vi "LTE_Example.vi"() -> ()   [LabVIEW 2016]
doc: "This example illustrates how to use the RFmxLTE APIs to configure the analyzer to do ModAcc measurement. You can use the Generator Basic example to generate the LTE signal before running this example."
uses:
  Source/SA/RFmxLTE/Typedefs/LTE ModAcc Configuration.ctl
  Source/SA/RFmxLTE/Typedefs/LTE ModAcc Results.ctl
  Source/SA/RFmxLTE/Typedefs/LTE ModAcc Component Carrier Results.ctl
  Source/SA/RFmxInstr/Typedefs/Instrument Configuration.ctl
  Source/Common/Local Oscillator Sharing Mode.ctl
  Source/Common/SA Common Configuration.ctl
  Source/SA/RFmxLTE/Typedefs/LTE Standard Configuration.ctl
  Source/SA/RFmxLTE/Typedefs/LTE Component Carrier Configuration.ctl
  Source/Common/SA Auto Level Configuration.ctl
  Source/SA/RFmxLTE/RFmxLTE.lvlib
  Source/SA/RFmxInstr/RFmxInstr.lvlib
  Source/Common/Common.lvlib
panel:
  out "error out":errorcluster
  out "ModAcc Results":T1
  in  "Tab Control":enum32{"Common", "Standard", "ModAcc"}(tab)
  in  "Resource Name":refnum<k15>="5840"
  in  "Common Configuration":T3={"Center Frequency (Hz)"=3500000000.0, "Reference Level (dBm)"=0.0, "External Attenuation (dB)"=0.0, "Trigger Enabled"=TRUE, "Digital Trigger Source"="PXI_Trig0", "Trigger Delay (s)"=0.0, "Selected Ports"=""} {"Trigger Delay (s)" format="%.2p"; "External Attenuation (dB)" format="%.2f"; "Reference Level (dBm)" format="%.2f"; "Center Frequency (Hz)" format="%.6p"}
  in  "Instrument Configuration":T4={"LO Sharing Mode"=enum."Automatic", "Frequency Reference Source"="PXI_Clk"}
  in  "Auto Level Configuration":T6={"Enabled"=TRUE, "Measurement Interval (s)"=0.01} {"Measurement Interval (s)" min=1e-06 max=100.0 format="%.2p"}
  in  "LTE Standard Configuration":T7={"Link Direction"=1, "Duplex Scheme"=0, "Uplink Downlink Configuration"=0, "Band"=1, "PUSCH Auto Resource Block Detection Enabled"=1, "Auto DMRS Detection Enabled"=1, "Downlink Auto Cell ID Detection Enabled"=0, "Component Carrier Configurations"=[{"Bandwidth (Hz)"=20000000.0, "Cell ID"=0, "PUSCH Modulation Type"=0, "PUSCH Resource Block Offset"=0, "PUSCH Number of Resource Blocks"=-1, "Downlink Test Model"=0}]} {"Downlink Auto Cell ID Detection Enabled" items=["False", "True"]; "Link Direction" items=["Downlink", "Uplink"]; "Auto DMRS Detection Enabled" items=["False", "True"]; "PUSCH Auto Resource Block Detection Enabled" items=["False", "True"]; "Component Carrier Configurations"."Downlink Test Model" items=["TM1.1", "TM1.2", "TM2", "TM 2a", "TM 3.1", "TM 3.2", "TM 3.3", "TM 3.1a"]; "Component Carrier Configurations"."PUSCH Modulation Type" items=["QPSK", "16 QAM", "64 QAM", "256 QAM", "1024 QAM"]; "Component Carrier Configurations"."Bandwidth (Hz)" items=["200.0 k"=200000.0, "1.4 M"=1400000.0, "3.0 M"=3000000.0, "5.0 M"=5000000.0, "10.0 M"=10000000.0, "15.0 M"=15000000.0, "20.0 M"=20000000.0]; "Uplink Downlink Configuration" items=["0", "1", "2", "3", "4", "5", "6"]; "Duplex Scheme" items=["FDD", "TDD", "LAA"]}
  in  "ModAcc Configuration":T9={"Synchronization Mode"=1, "Measurement Offset"=0, "Measurement Length"=1, "EVM Unit"=0, "Averaging Enabled"=0, "Averaging Count"=10} {"Averaging Enabled" items=["Percentage", "dB"]; "EVM Unit" items=["Percentage", "dB"]; "Synchronization Mode" items=["Frame", "Slot", "Marker"]}
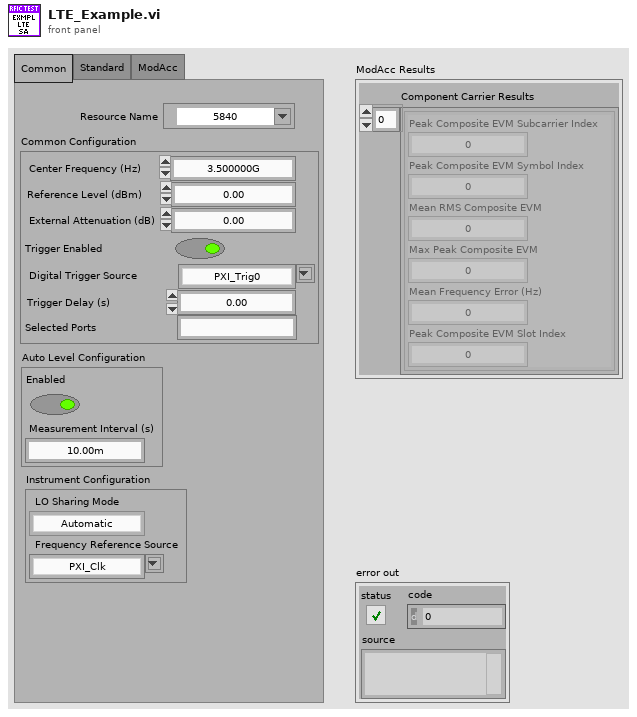
[diagram p1: front panel]
types:
  T1 = typedef "RFmxLTE.lvlib/LTE ModAcc Results.ctl" = cluster{"Component Carrier Results":T2[]}
  T2 = typedef "RFmxLTE.lvlib/LTE ModAcc Component Carrier Results.ctl" = cluster{"Peak Composite EVM Subcarrier Index":i32, "Peak Composite EVM Symbol Index":i32, "Mean RMS Composite EVM":dbl, "Max Peak Composite EVM":dbl, "Mean Frequency Error (Hz)":dbl, "Peak Composite EVM Slot Index":i32}
  T3 = typedef "Common.lvlib/SA Common Configuration.ctl" = cluster{"Center Frequency (Hz)":dbl, "Reference Level (dBm)":dbl, "External Attenuation (dB)":dbl, "Trigger Enabled":bool, "Digital Trigger Source":string, "Trigger Delay (s)":dbl, "Selected Ports":string}
  T4 = typedef "RFmxInstr.lvlib/Instrument Configuration.ctl" = cluster{"LO Sharing Mode":T5, "Frequency Reference Source":string}
  T5 = typedef "Common.lvlib/Local Oscillator Sharing Mode.ctl" = enum16{"Automatic", "None"}
  T6 = typedef "Common.lvlib/SA Auto Level Configuration.ctl" = cluster{"Enabled":bool, "Measurement Interval (s)":dbl}
  T7 = typedef "RFmxLTE.lvlib/LTE Standard Configuration.ctl" = cluster{"Link Direction":i32, "Duplex Scheme":i32, "Uplink Downlink Configuration":i32, "Band":i32, "PUSCH Auto Resource Block Detection Enabled":i32, "Auto DMRS Detection Enabled":i32, "Downlink Auto Cell ID Detection Enabled":i32, "Component Carrier Configurations":T8[]}
  T8 = typedef "RFmxLTE.lvlib/LTE Component Carrier Configuration.ctl" = cluster{"Bandwidth (Hz)":dbl, "Cell ID":i32, "PUSCH Modulation Type":i32, "PUSCH Resource Block Offset":i32, "PUSCH Number of Resource Blocks":i32, "Downlink Test Model":i32}
  T9 = typedef "RFmxLTE.lvlib/LTE ModAcc Configuration.ctl" = cluster{"Synchronization Mode":i32, "Measurement Offset":i32, "Measurement Length":i32, "EVM Unit":i32, "Averaging Enabled":i32, "Averaging Count":i32}
  T10 = enum16{"ACP", "CHP", "ModAcc", "OBW", "SEM", "PVT", "SlotPhase", "SlotPower"}[]
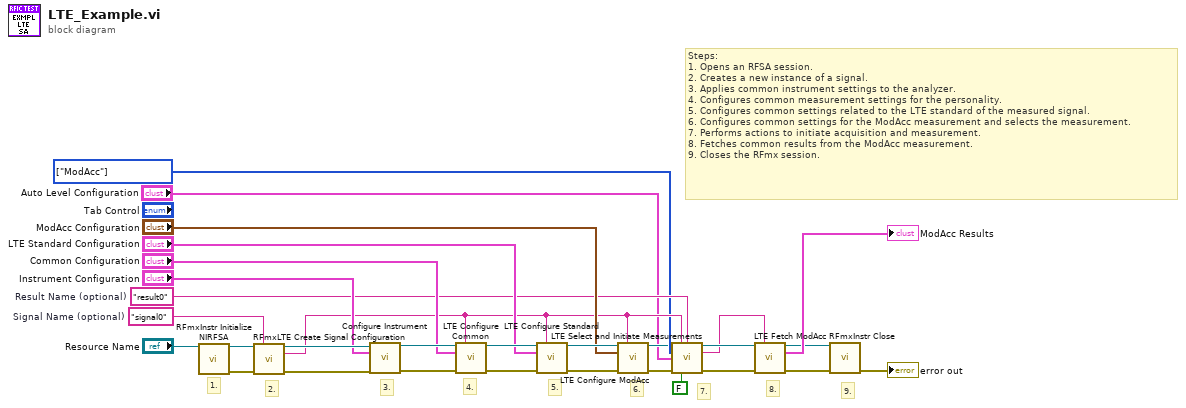
[diagram p0: block diagram]
diagram:
  w10 = T10 [enum."ModAcc"] items=["ACP", "CHP", "ModAcc", "OBW", "SEM", "PVT", "SlotPhase", "SlotPower"] ("Measurements")
  w11 = "result0"  # Result Name (optional)
  w20 = "signal0"  # Signal Name (optional)
  # "Steps: \n1. Opens an RFSA session.\n2. Creates a new instance of a signal.\n3. Applies common instrument settings to the analyzer.\n4. Configures common measurement settings for the personality.\n5. Configures common settings related to the LTE standard of the measured signal.\n6. Configures common settings for the ModAcc measurement and selects the measurement.\n7. Performs actions to initiate acquisition and measurement. \n8. Fetches common results from the ModAcc measurement.\n9. Closes the RFmx session."
  # "9."
  # "8."
  # "7."
  # "6."
  # "5."
  # "4."
  # "3."
  # "2."
  # "1."
  n1 = call <vilib>:"RFmxInstr Initialize NIRFSA.vi"("Resource Name"="Resource Name") -> ("Instrument Handle Out"=w21:refnum<k21>, "error out"=w28:errorcluster)  [unwired: 12 in, 1 out]
  n2 = call <vilib>:"RFmxLTE Create Signal Configuration.vi"("Instrument Handle In"=w21, "Signal Name"=w20, "error in (no error)"=w28) -> ("Instrument Handle Out"=w19:refnum<k21>, "Selector String Out"=w12:string, "error out"=w3:errorcluster)  [unwired: 10 in]
  n3 = call "Configure Instrument.vi"("Instrument Handle In"=w19, "Instrument Configuration"="Instrument Configuration", "error in (no error)"=w3) -> ("Instrument Handle Out"=w18:refnum<k21>, "error out"=w2:errorcluster)  [unwired: 11 in]
  n4 = call "LTE Configure Common.vi"("RFmx Handle In"=w18, "Selector String"=w12, "Common Configuration"="Common Configuration", "error in (no error)"=w2) -> ("RFmx Handle Out"=w30:refnum<k21>, "error out"=w29:errorcluster)  [unwired: 10 in]
  n5 = call "LTE Configure Standard.vi"("RFmx Handle In"=w30, "Selector String"=w12, "LTE Standard Configuration"="LTE Standard Configuration", "error in (no error)"=w29) -> ("RFmx Handle Out"=w26:refnum<k21>, "error out"=w25:errorcluster)  [unwired: 10 in]
  n6 = call "LTE Configure ModAcc.vi"("RFmx Handle In"=w26, "Selector String"=w12, "ModAcc Configuration"="ModAcc Configuration", "error in (no error)"=w25) -> ("RFmx Handle Out"=w7:refnum<k21>, "error out"=w4:errorcluster)  [unwired: 10 in]
  n7 = call "LTE Select and Initiate Measurements.vi"("Instrument Handle In"=w7, "Selector String"=w12, "Result Name"=w11, "Measurements"=w10, "Auto Level Configuration"="Auto Level Configuration", "error in (no error)"=w4, "Enable All Traces (F)"=FALSE) -> ("Instrument Handle Out"=w14:refnum<k21>, "Selector String Out"=w9:string, "error out"=w13:errorcluster)  [unwired: 6 in]
  n8 = call "LTE Fetch ModAcc.vi"("RFmx Handle In"=w14, "Selector String"=w9, "error in (no error)"=w13) -> ("RFmx Handle Out"=w6:refnum<k21>, "ModAcc Results"=→"ModAcc Results":T1, "error out"=w5:errorcluster)  [unwired: 10 in]
  n9 = call <vilib>:"RFmxInstr Close.vi"("Instrument Handle In"=w6, "error in (no error)"=w5) -> ("error out"=→"error out":errorcluster)  [unwired: 13 in]
